vi "Script.vi"(8 "error in":errorcluster, 11 "Actor in":refnum<class "Actor.lvclass">) -> (0 "error out":errorcluster, 3 "Actor out":refnum<class "Actor.lvclass">)   [LabVIEW 2020, in "_Rescript.lvlib" / "Actor.lvlib" / "Actor.lvclass"]
uses:
  Actor.lvclass
  Actor.lvclass/Actor.ctl
  Script Con And Wire.vi
  Find Pane.vi
  Terminal Attributes Descending Order.vi
  SubVI Terminals.vi
  <vilib>/Utility/traverseref.llb/TRef Find Object By Label.vi
  Script Control To ConPane.vi
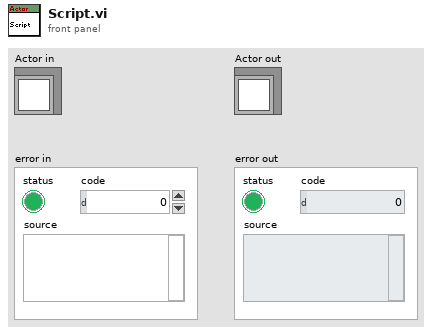
[diagram p1: front panel]
types:
  T1 = typedef "_Rescript.lvlib/Actor.lvlib/Actor.lvclass/Name Actor.ctl" = cluster{"Init Actor VI (Class)":refnum<vi>, "Init Actor VI (Lib)":refnum<vi>, "Terminal Attributes (Init)":T2}
  T2 = typedef "_Rescript.lvlib/Terminal Attributes.ctl" = map{i32, T3}
  T3 = typedef "_Rescript.lvlib/Attributes.ctl" = cluster{"Control":refnum<vi>, "Wire Rule":enum16{"Invalid Wire Rule", "Required", "Recommended", "Optional", "Dynamic Dispatch"}}
  T4 = typedef "_Rescript.lvlib/Actor.lvlib/Actor.lvclass/Name.ctl" = cluster{"Init Actor VI (Lib)":refnum<vi>}
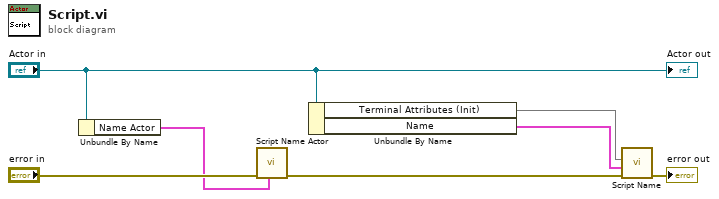
[diagram p0: block diagram]
diagram:
  n1 = Unbundle By Name("Actor in") -> ("Name Actor"=w3:T1)
  n2 = call "Script Name Actor.vi"("Name Actor"=w3, "error in"="error in") -> ("error out"=w7:errorcluster)  [unwired: 9 in]
  n3 = Unbundle By Name("Actor in") -> ("Terminal Attributes (Init)"=w1:T2, "Name"=w2:T4)
  n4 = call "Script Name.vi"("error in"=w7, "Name"=w2, "Name Actor.Terminal Attributes (Init)"=w1) -> ("error out"=→"error out":errorcluster)  [unwired: 8 in]
  "Actor out" <- "Actor in"
